vi "VIH ProjFile - Create.vi"(8 "error in":errorcluster) -> (0 "error out":errorcluster, 3 "Project":T1)   [LabVIEW 2014]
doc: "::: VI Helpeks :::\nCopyright (c) 2000-2026 Konstantin Shifershteyn. All rights reserved."
uses:
  <vilib>/xml/NI_XML.lvlib
  <resource>/objmgr/DOMUserDefRef.rc
panel:
  # "VI Helpeks\nCopyright (c) 2012-2026 Konstantin Shifershteyn"
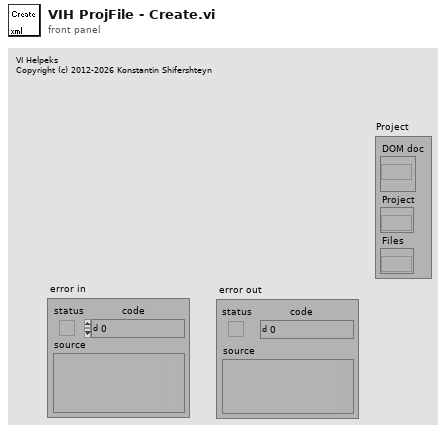
[diagram p1: front panel]
types:
  T1 = cluster{"DOM doc":refnum<k20>, "Project":refnum<k20>, "Files":refnum<k20>}
  T2 = cluster{"DOM document out":refnum<k20>, "New Element":refnum<k20>, "New Element":refnum<k20>}
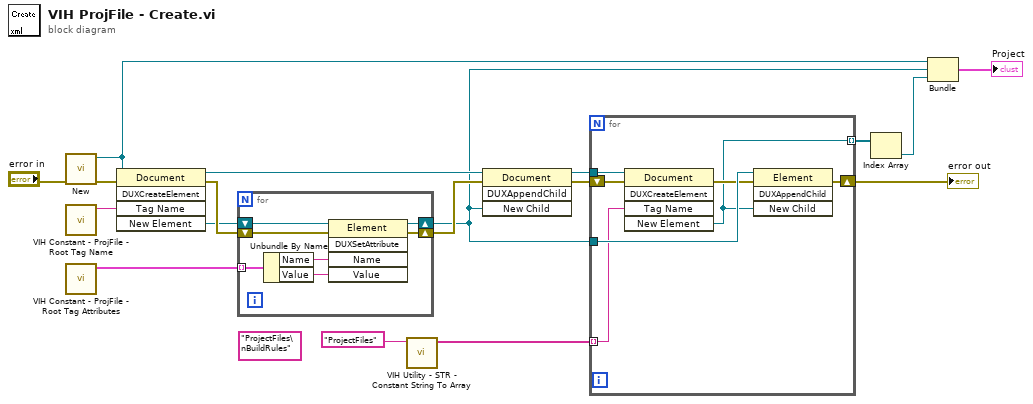
[diagram p0: block diagram]
diagram:
  (unwired) "ProjectFiles\nBuildRules" ("Tag Name")
  n1 = call <vilib>:"New.vi"("error in (no error)"="error in") -> ("error out"=w18:errorcluster, "DOM document out"=w8:refnum<k20>)  [unwired: 7 in]
  n2 = call "VIH Constant - ProjFile - Root Tag Name.vi"() -> ("Tag Name"=w2:string)  [unwired: 11 in]
  n3 = call "VIH Constant - ProjFile - Root Tag Attributes.vi"() -> ("Root Tag Attributes"=w1:cluster{"Name":string, "Value":string}[])  [unwired: 11 in]
  n4 = invoke class="Document" method="DUXCreateElement"(reference=w8, error in=w18, "Tag Name"=w2) -> (reference out=w15:refnum<k20>, error out=w17:errorcluster, "New Element"=w16:refnum<k20>)  [unwired: 2 in, 2 out]
  n5 = for {
    shift-right: [w23] -> w14
    shift-left: w17 -> [w25]
    shift-right: [w22] -> w6
    shift-left: w16 -> [w24]
    tunnel: w1 -> [w21] mode=indexing
    n6 = Unbundle By Name(w21) -> ("Name"=w20:string, "Value"=w19:string)
    n7 = invoke class="Element" method="DUXSetAttribute"(reference=w24, error in=w25, "Name"=w20, "Value"=w19) -> (reference out=w22:refnum<k20>, error out=w23:errorcluster)  [unwired: 1 in, 3 out]
  }
  n8 = call "VIH Utility - STR - Constant String To Array.vi"("String in"="ProjectFiles" ("Tag Name")) -> ("Array out"=w3:string[])  [unwired: 10 in]
  n9 = invoke class="Document" method="DUXAppendChild"(reference=w15, error in=w14, "New Child"=w6) -> (reference out=w12:refnum<k20>, error out=w11:errorcluster)  [unwired: 1 in, 2 out]
  n10 = for {
    tunnel: w12 -> [w32]
    shift-right: [w29] -> w10
    shift-left: w11 -> [w31]
    tunnel: w6 -> [w30]
    tunnel: w3 -> [w28] mode=indexing
    tunnel: [w26] -> w9 mode=indexing
    n11 = invoke class="Document" method="DUXCreateElement"(reference=w32, error in=w31, "Tag Name"=w28) -> (error out=w27:errorcluster, "New Element"=w26:refnum<k20>)  [unwired: 2 in, 3 out]
    n12 = invoke class="Element" method="DUXAppendChild"(reference=w30, error in=w27, "New Child"=w26) -> (error out=w29:errorcluster)  [unwired: 1 in, 3 out]
  }
  "error out" <- w10
  n13 = Index Array(array=w9) -> (element=w5:refnum<k20>)  [unwired: 1 in]
  n14 = Bundle("DOM document out"=w8, "New Element"=w6, "New Element"=w5) -> (→"Project":T2)  [unwired: 1 in]
